vi "set Operation Band.vi"(8 "error in (no error)":errorcluster, 9 "Selected CC Argements":T1, 10 "Operation Band":u32, 11 "NR in":refnum<class "NR.lvclass">) -> (0 "error out":errorcluster, 3 "NR out":refnum<class "NR.lvclass">)   [LabVIEW 2023, in "ANRITSU Call Box.lvlib" / "NR.lvclass"]
uses:
  NR.lvclass
  NR.lvclass/NR.ctl
  Type Definition/NR Selected CC Type Arguments.ctl
  ANRITSU Call Box.lvlib
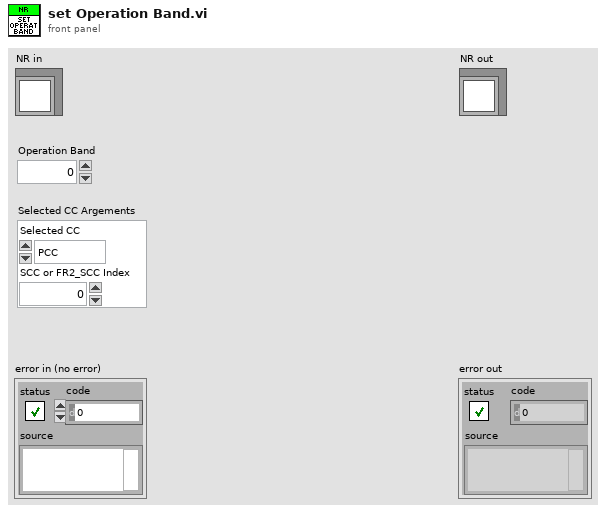
[diagram p1: front panel]
types:
  T1 = typedef "ANRITSU Call Box.lvlib/NR Selected CC Type Arguments.ctl" = cluster{"Selected CC":enum16{"PCC", "SCC", "FR2_PCC", "FR2_SCC"}, "SCC or FR2_SCC Index":u32}
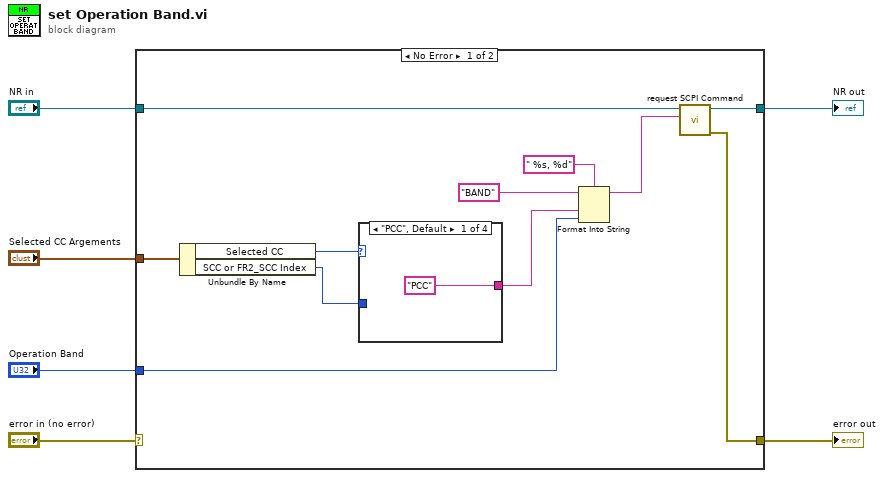
[diagram p0: block diagram]
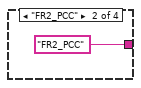
[diagram p2: hidden frame]
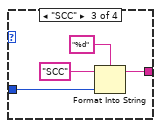
[diagram p3: hidden frame]
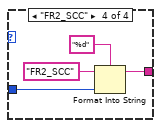
[diagram p4: hidden frame]
diagram:
  n1 = case shown="No Error" "error in (no error)" {
    selector: "error in (no error)" -> [_ w28]
    tunnel: "NR in" -> [w10 w29]
    tunnel: [w8 w29] -> w5
    tunnel: [w7 w28] -> w4
    tunnel: "Selected CC Argements" -> [w17 _]
    tunnel: "Operation Band" -> [w11 _]
    frame No Error {
      n2 = Unbundle By Name(w17) -> ("Selected CC"=w16:enum16{"PCC", "SCC", "FR2_PCC", "FR2_SCC"}, "SCC or FR2_SCC Index"=w15:u32)
      n3 = case shown="\"PCC\", Default" w16 {
        tunnel: ["PCC" "FR2_PCC" w20 w24] -> w12
        tunnel: w15 -> [_ _ w21 w25]
        frame "PCC", Default {
        }
        frame "FR2_PCC" {
        }
        frame "SCC" {
          n4 = Format Into String(format string="%d", initial string="SCC", w21) -> (resulting string=w20:string)  [unwired: 1 in, 1 out]
        }
        frame "FR2_SCC" {
          n5 = Format Into String(format string="%d", initial string="FR2_SCC", w25) -> (resulting string=w24:string)  [unwired: 1 in, 1 out]
        }
      }
      n6 = Format Into String(format string=" %s, %d", initial string="BAND", w12, w11) -> (resulting string=w9:string)  [unwired: 1 in, 1 out]
      n7 = call "request SCPI Command.vi"("SCPI Command"=w9, "NR in"=w10) -> ("error out"=w7:errorcluster, "NR out"=w8:refnum<class "NR.lvclass">)  [unwired: 8 in]
    }
    frame Error {
    }
  }
  "error out" <- w4
  "NR out" <- w5
